vi "Repeat.vi"(11 "CSM Name":string="Repeat") -> ()   [LabVIEW 2026, in "UI-温度控制.lvlib" / "Repeat.lvlib"]
uses:
  Repeat.lvlib
  Supports/Repeat Steps.ctl
  Supports/Repeating States.ctl
  <userlib>/_NEVSTOP/Communicable State Machine(CSM)/_Polymophic/CSM - Filter Duplicated Lines.vi
  816fba94-53db-458f-9fde-c2796c7a1569.vi
  ba2d9a0e-10df-4741-bda9-2194bb22ae09.vi
  ed04b07b-11fd-4180-b0fa-2f6e8442eecc.vi
  <userlib>/_NEVSTOP/Communicable State Machine(CSM)/_Polymophic/Build Synchronous Message with Arguments.vi
  63e03b33-849f-44e3-ac5e-f4abb9122a72.vi
  801019de-d43e-4a0a-86cc-ff4224036546.vi
  2ffd62ee-fbfc-4690-b0a4-2e8231dd450f.vi
  1f220b95-32e7-4906-b34d-524106bf87b5.vi
  b2c443a6-884a-417f-a1f3-5b041c9b1280.vi
  <userlib>/_NEVSTOP/Communicable State Machine(CSM)/AdvanceAPI/CSM - Compact Multiple States.vi
  <userlib>/_NEVSTOP/Communicable State Machine(CSM)/AdvanceAPI/CSM - Break Down Multiple States String.vi
  <userlib>/_NEVSTOP/Communicable State Machine(CSM)/_Shared/Remove Comments from Single-line.vi
  <userlib>/_NEVSTOP/Communicable State Machine(CSM)/_Shared/Split Single-line Message.vi
  <userlib>/_NEVSTOP/Communicable State Machine(CSM)/_Shared/Trim Single-line Text.vi
  <userlib>/_NEVSTOP/Communicable State Machine(CSM)/AdvanceAPI/CSM - Revert Arguments-Safe String.vi
  <userlib>/_NEVSTOP/Communicable State Machine(CSM)/AdvanceAPI/CSM - Make String Arguments Safe.vi
  <userlib>/_NEVSTOP/Communicable State Machine(CSM)/_Support/Message/Parse State with Arguments String.vi
  <userlib>/_NEVSTOP/Communicable State Machine(CSM)/AdvanceAPI/CSM - Keywords.vi
  <userlib>/_NEVSTOP/Communicable State Machine(CSM)/addons/API-String-Arugments-Support/_Support/Convert API String Arguments to Data(variant).vi
  <userlib>/_NEVSTOP/Communicable State Machine(CSM)/addons/API-String-Arugments-Support/_Support/Data To API String Arguments.vi
  <userlib>/_NEVSTOP/Communicable State Machine(CSM)/Communicable State Machine.lvlib
  <userlib>/_NEVSTOP/Communicable State Machine(CSM)/addons/Loop-Support/CSM Loop Support.lvlib
  <userlib>/_NEVSTOP/Communicable State Machine(CSM)/addons/INI-Static-Variable-Support/INI-Static-Variable-Support.lvlib
panel:
  in  "运行次数":dbl=inf format="%#.0f"
  out "当前次数":i32
  in  "通道选择":enum32{"1", "2", "1&2"}(radio)
  in  "循环开始":bool
  in  "步骤":T1=[{"控制温度"=25.0, "时长(s)"=600.0, "进度"=0.0, "温控开关"=FALSE}, {"控制温度"=25.0, "时长(s)"=600.0, "进度"=0.0, "温控开关"=FALSE}, {"控制温度"=25.0, "时长(s)"=600.0, "进度"=0.0, "温控开关"=FALSE}, {"控制温度"=25.0, "时长(s)"=600.0, "进度"=0.0, "温控开关"=FALSE}] {"进度" scale=0.0..1.0; "控制温度" format="%.2g"}
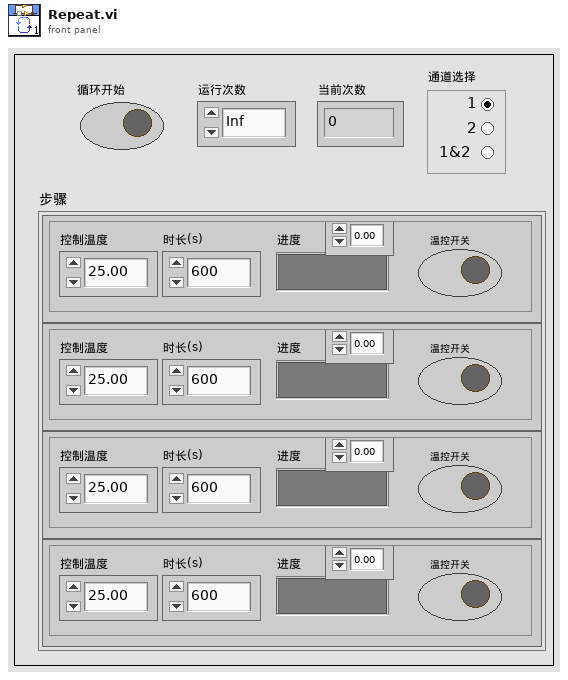
[diagram p1: front panel]
types:
  T1 = typedef "UI-温度控制.lvlib/Repeat Steps.ctl" = cluster{"控制温度":dbl, "时长(s)":dbl, "进度":dbl, "温控开关":bool}[]
  T2 = enum32{"Invalid", "Standard", "Closed", "Hidden", "Minimized", "Maximized"}
  T3 = enum32{"invalid app kind", "Development System", "Run Time System", "Student Edition", "Embedded LabVIEW", "Evaluation", "Custom"}
  T4 = typedef "UI-温度控制.lvlib/Repeat.lvlib/Repeating States.ctl" = enum16{"Idle", "Repeating", "Error"}
  T5 = typedef "Communicable State Machine.lvlib/_CSM_Response Source Message.ctl" = cluster{"‘State":string, "’Arguments":string, "’Error":errorcluster}
  T6 = cluster{"Current VI Reference":refnum<vi>, "Close Panel on Exit?":bool}
  T7 = cluster{"Core":cluster{"Current VI Reference":refnum<vi>, "Close Panel on Exit?":bool}, "State":T4, "Repeat":cluster{"温控步骤开始时间":timestamp, "温控步骤索引":i32[], "下一步？":bool}, "CSM Name":string, "INI Path":path}
  T8 = cluster{"温控步骤开始时间":timestamp, "温控步骤索引":i32[], "下一步？":bool}
  T9 = cluster{"控制温度":dbl, "时长(s)":dbl, "进度":dbl, "温控开关":bool}
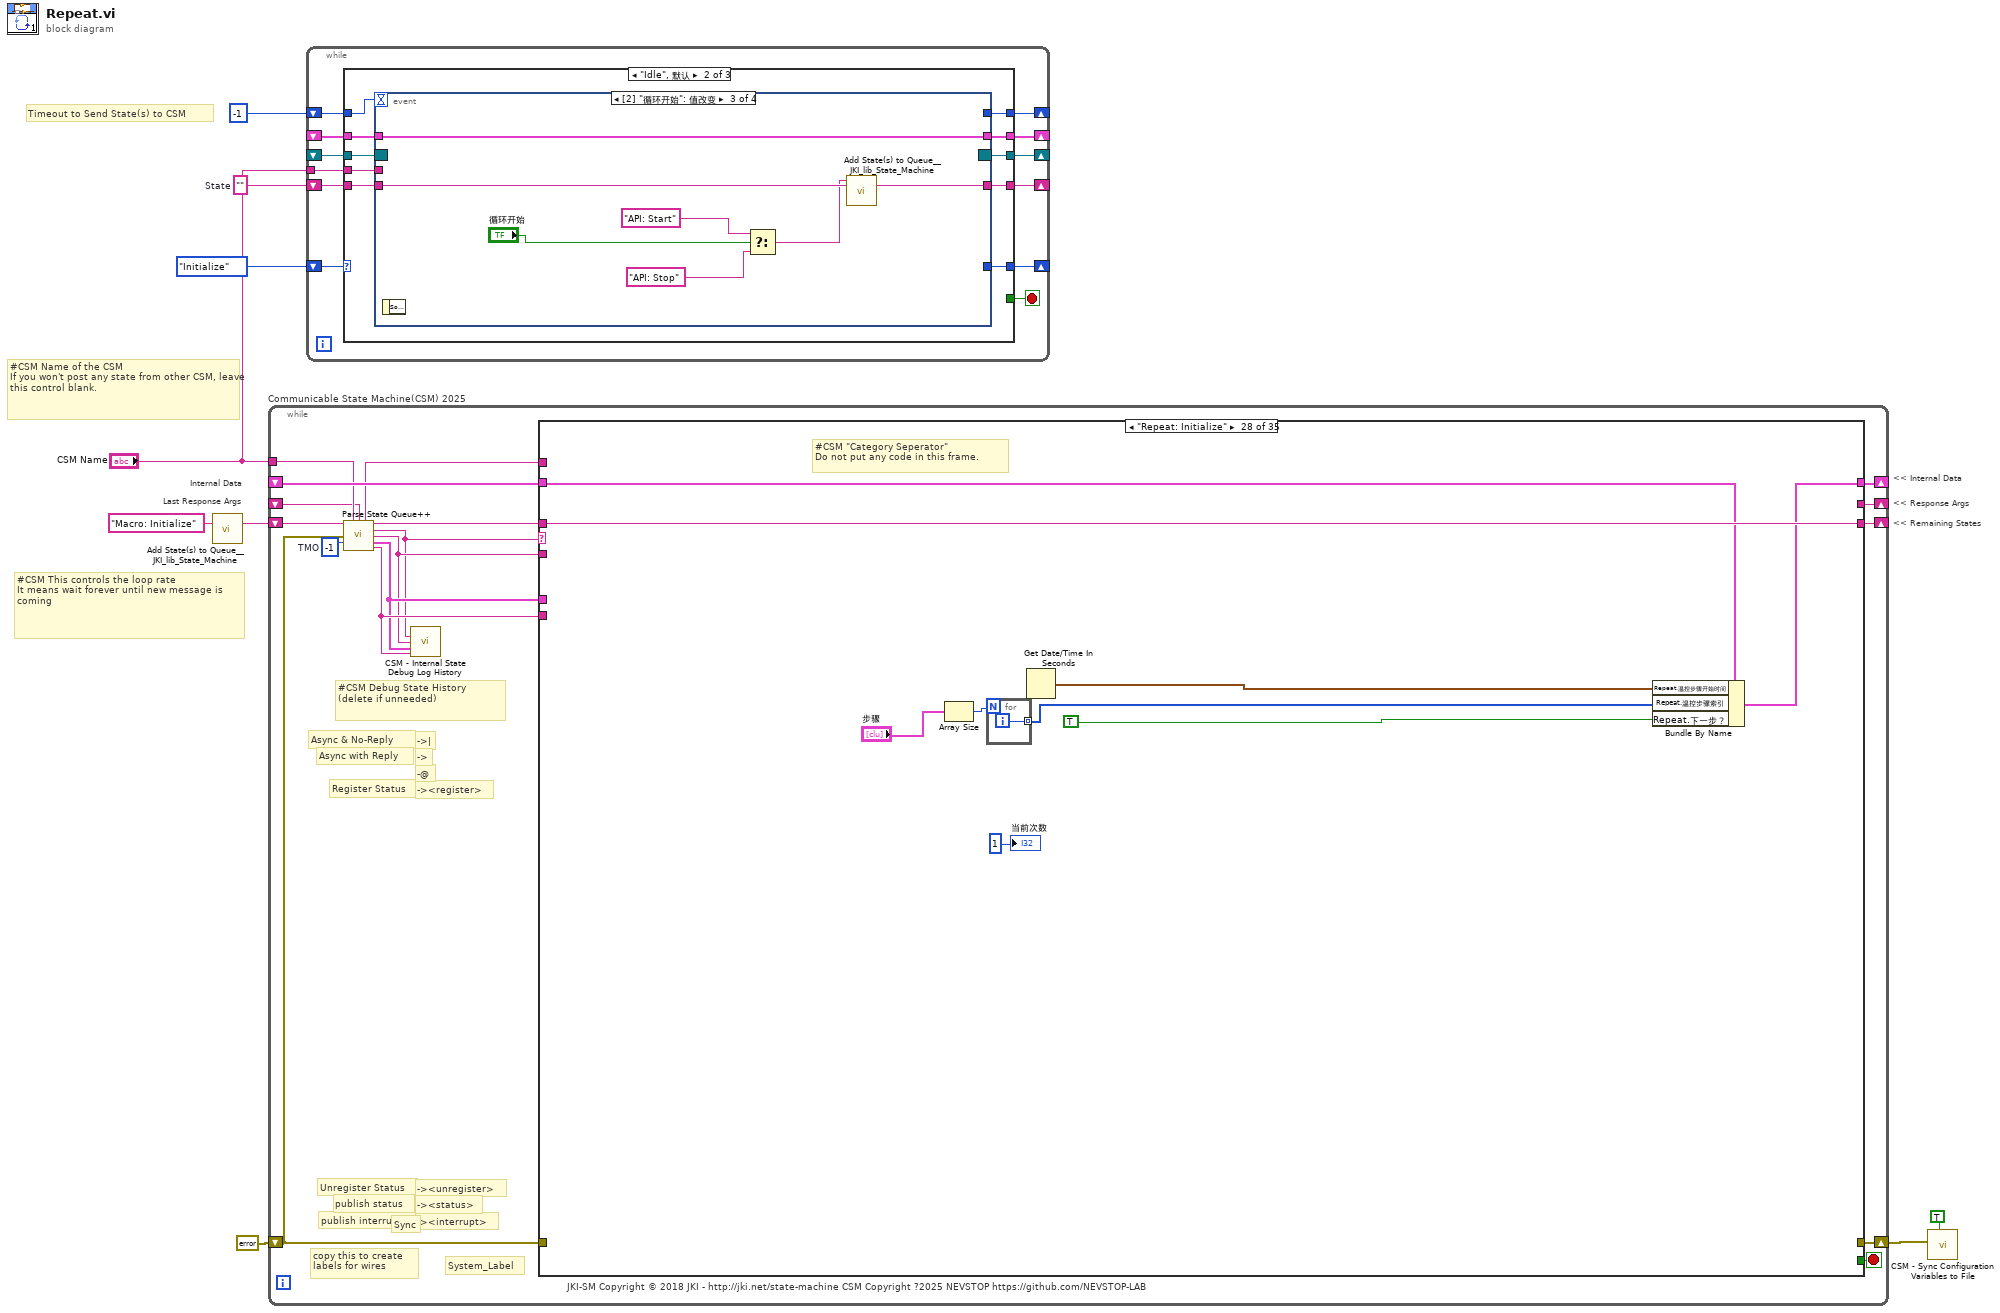
[diagram p0: block diagram]
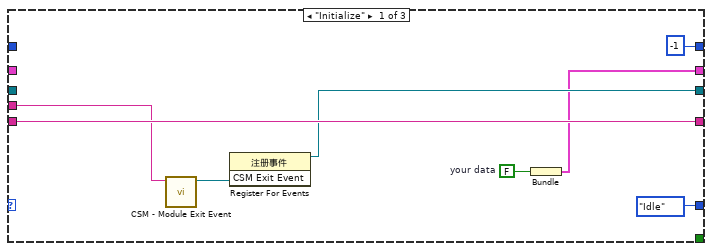
[diagram p2: hidden frame]
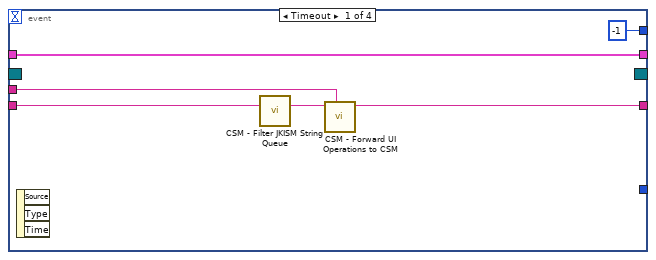
[diagram p3: hidden frame]
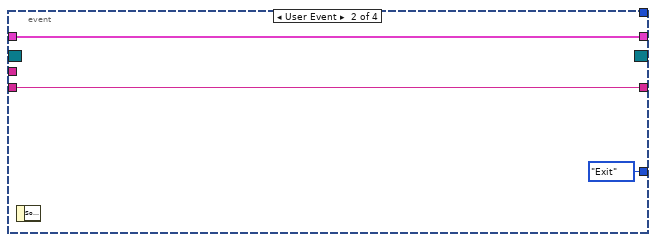
[diagram p4: hidden frame]
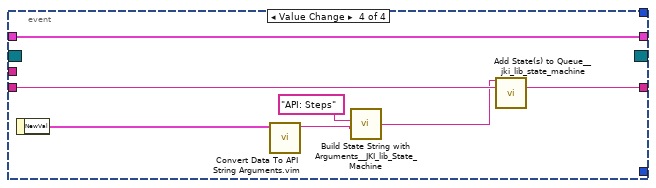
[diagram p5: hidden frame]
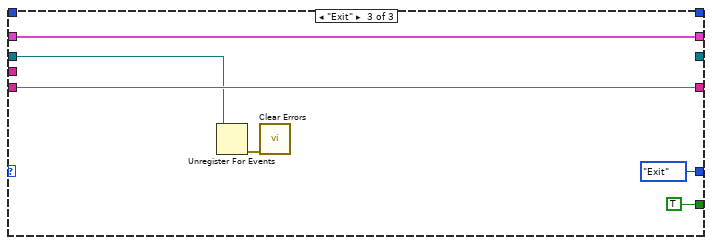
[diagram p6: hidden frame]
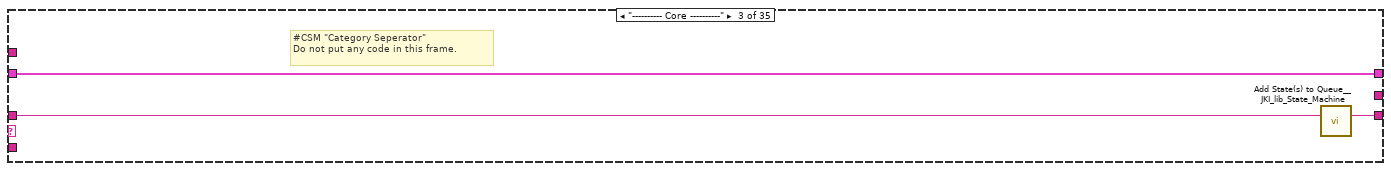
[diagram p9: hidden frame]
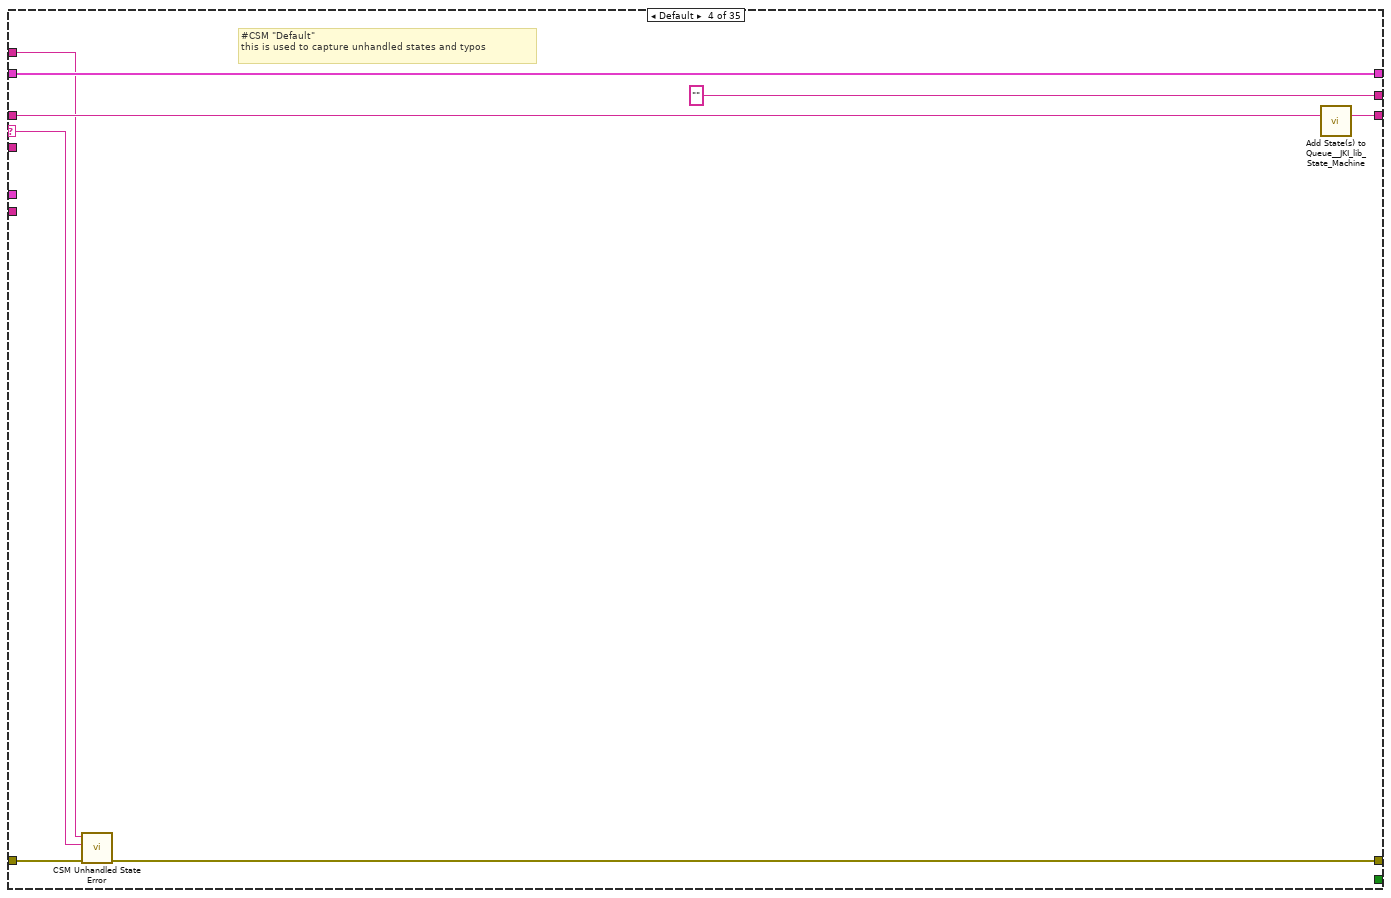
[diagram p10: hidden frame]
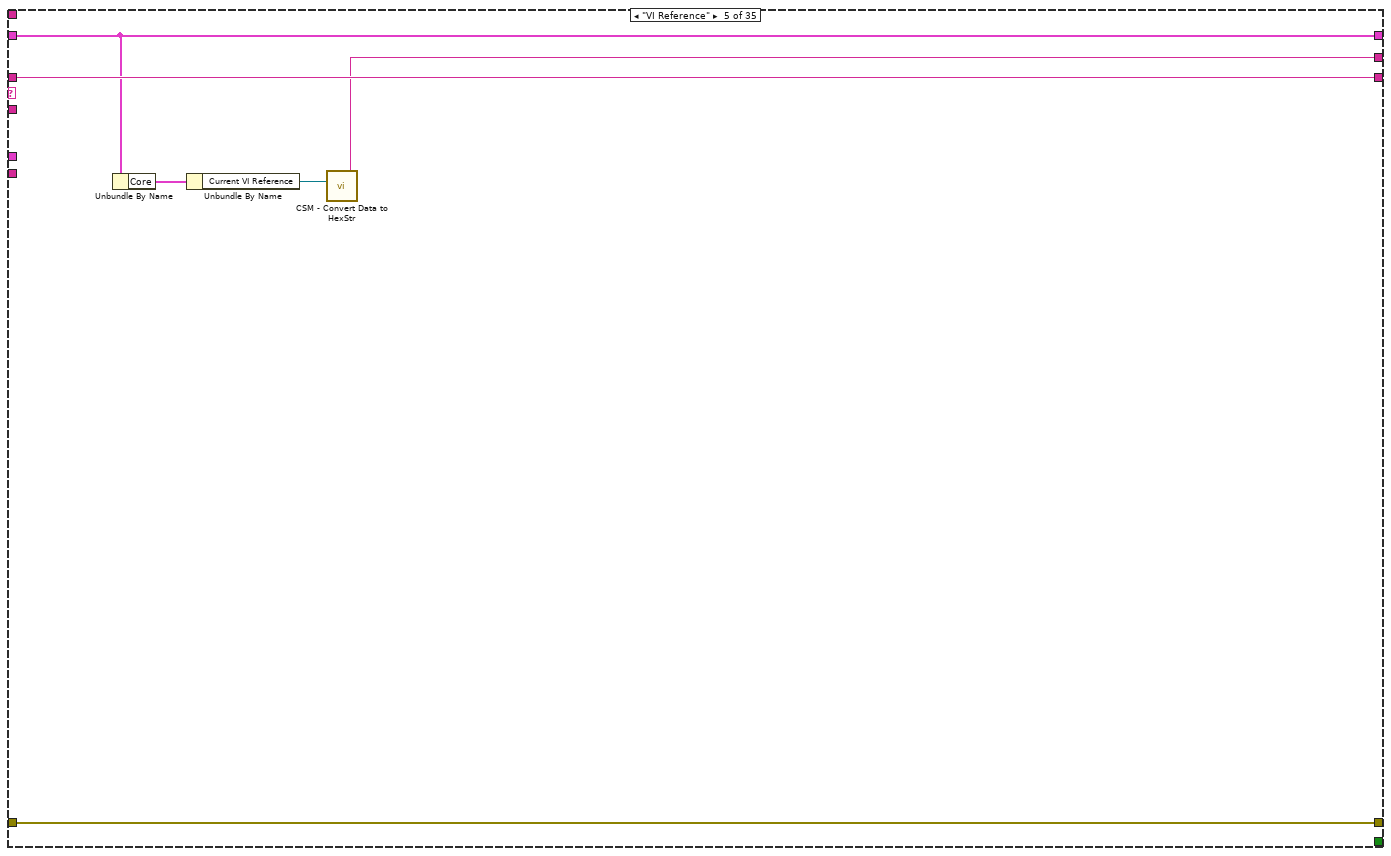
[diagram p11: hidden frame]
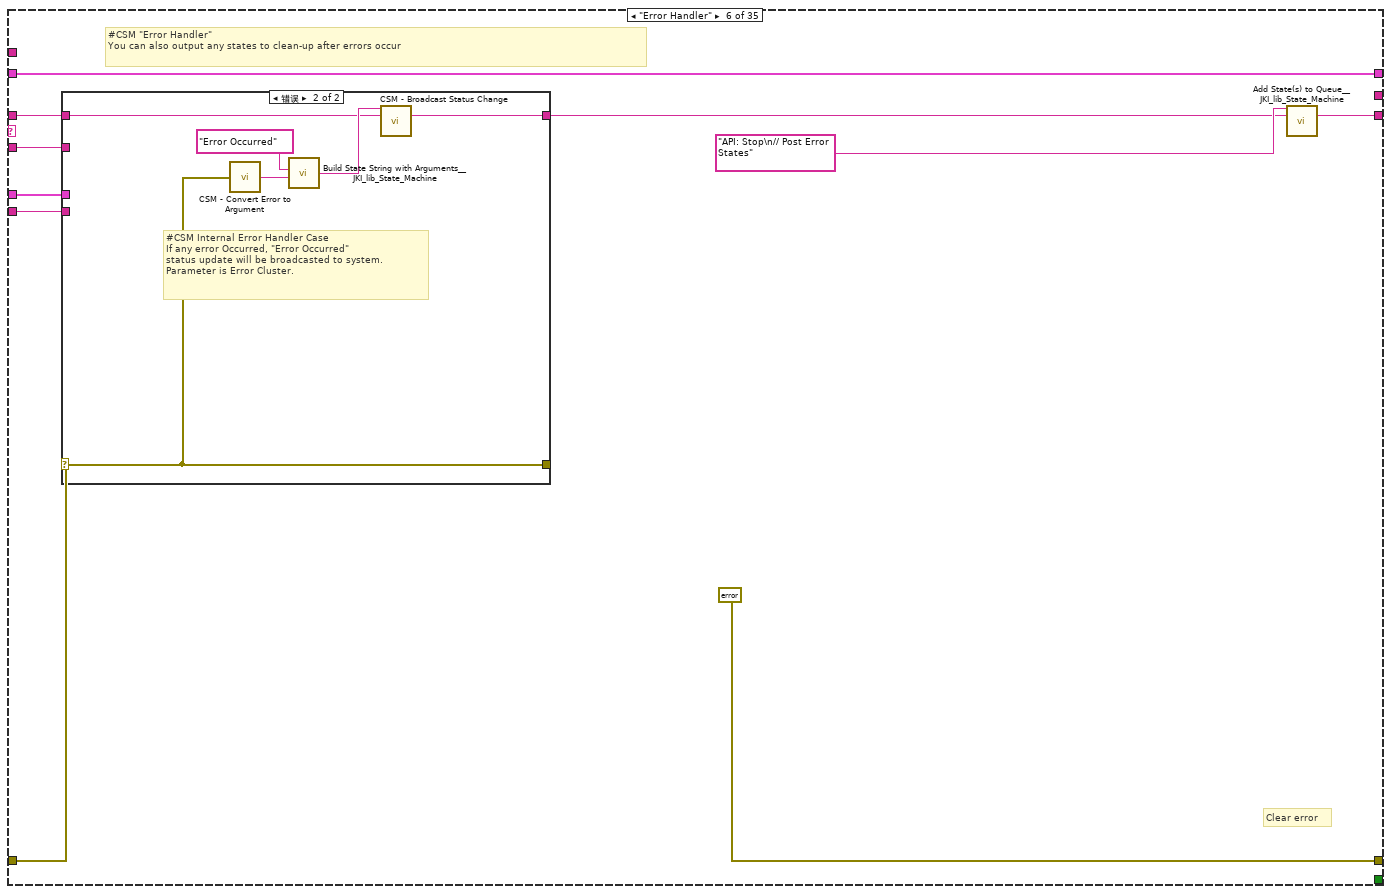
[diagram p12: hidden frame]
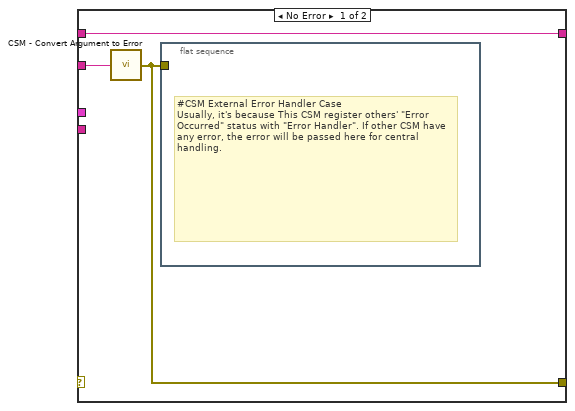
[diagram p13: hidden frame]
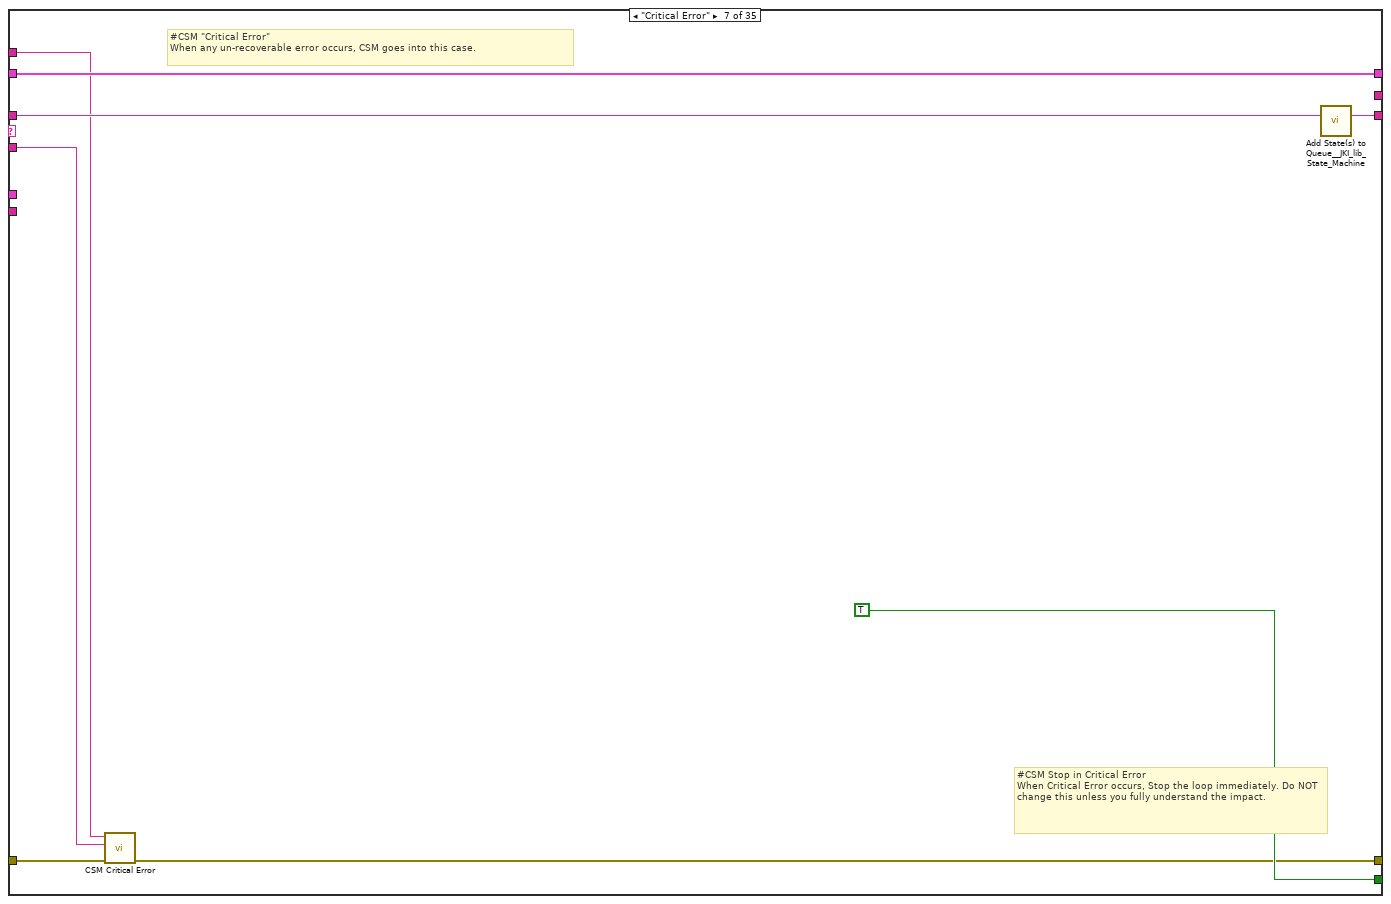
[diagram p14: hidden frame]
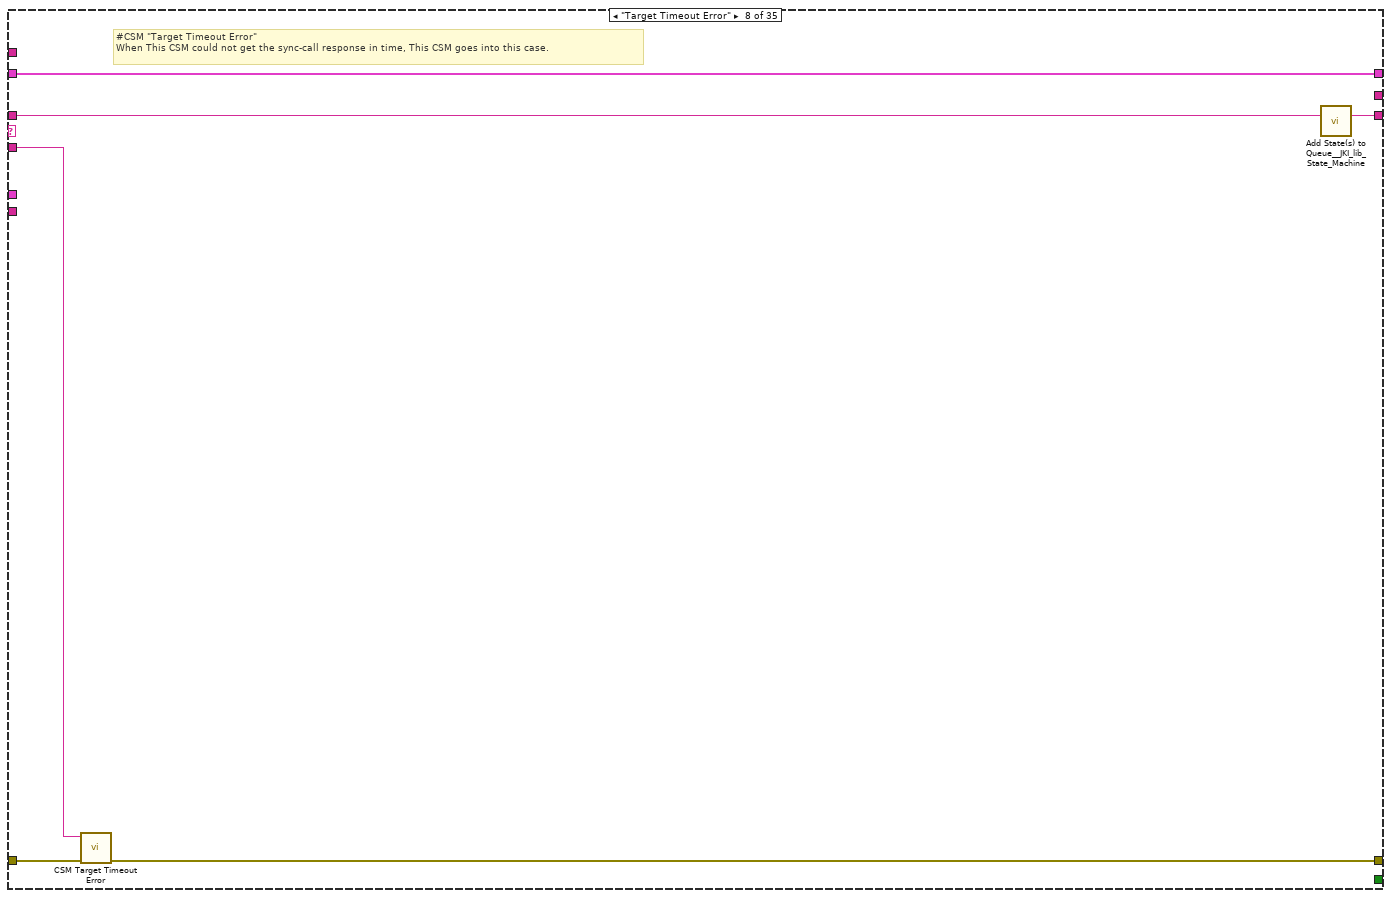
[diagram p15: hidden frame]
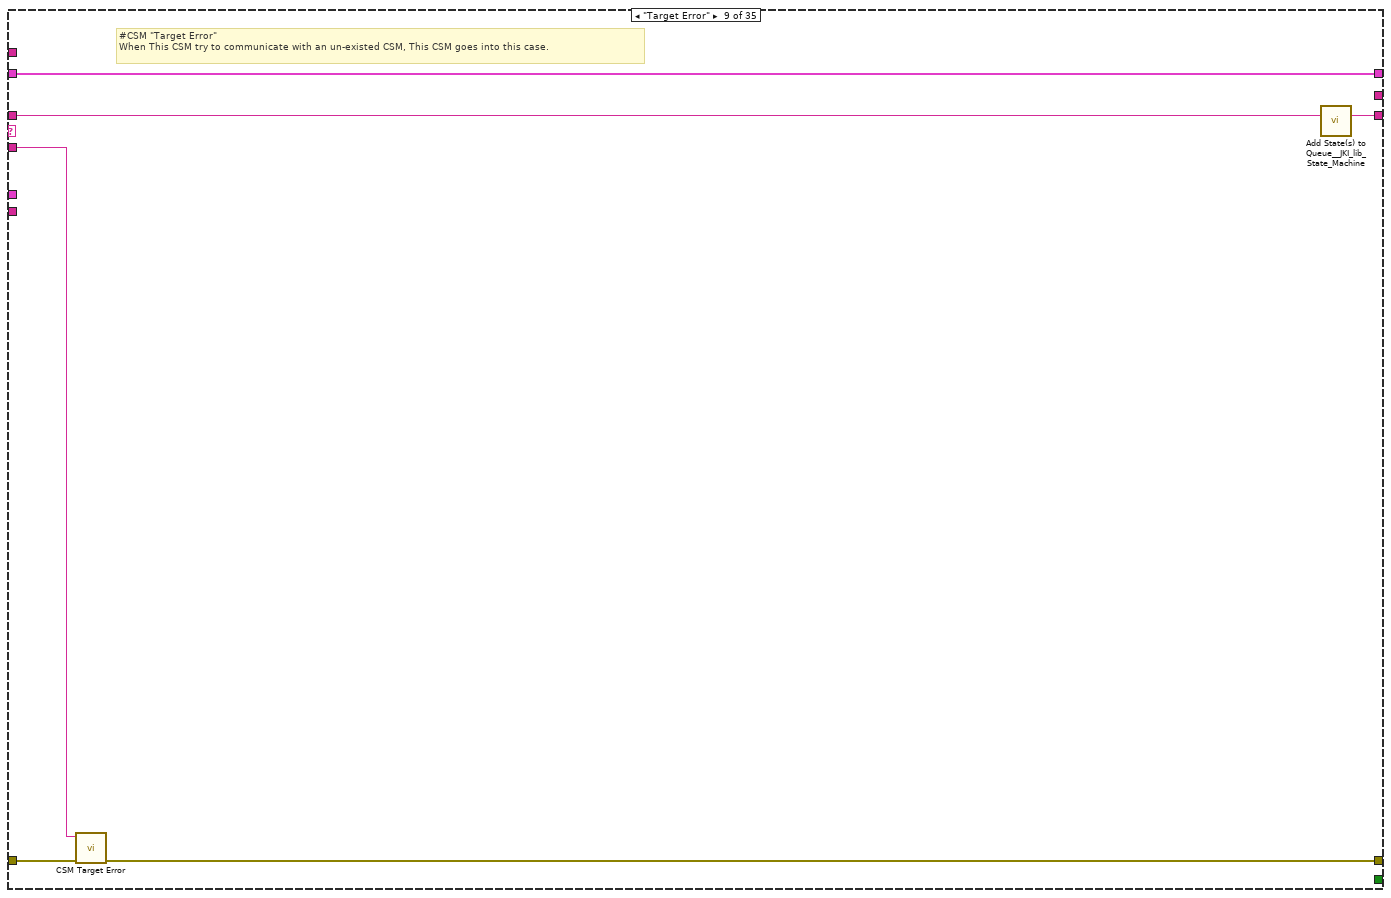
[diagram p16: hidden frame]
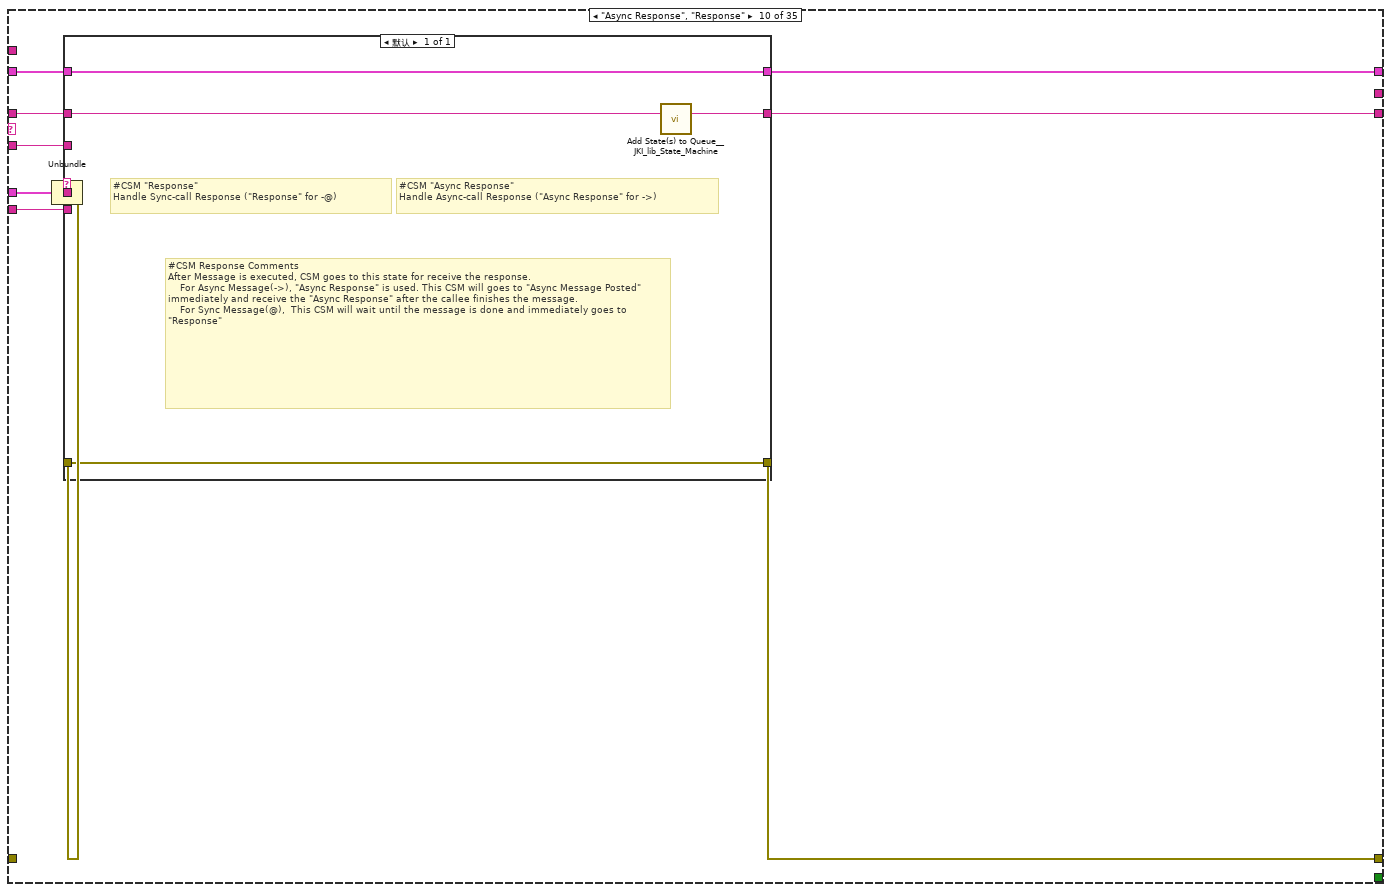
[diagram p17: hidden frame]
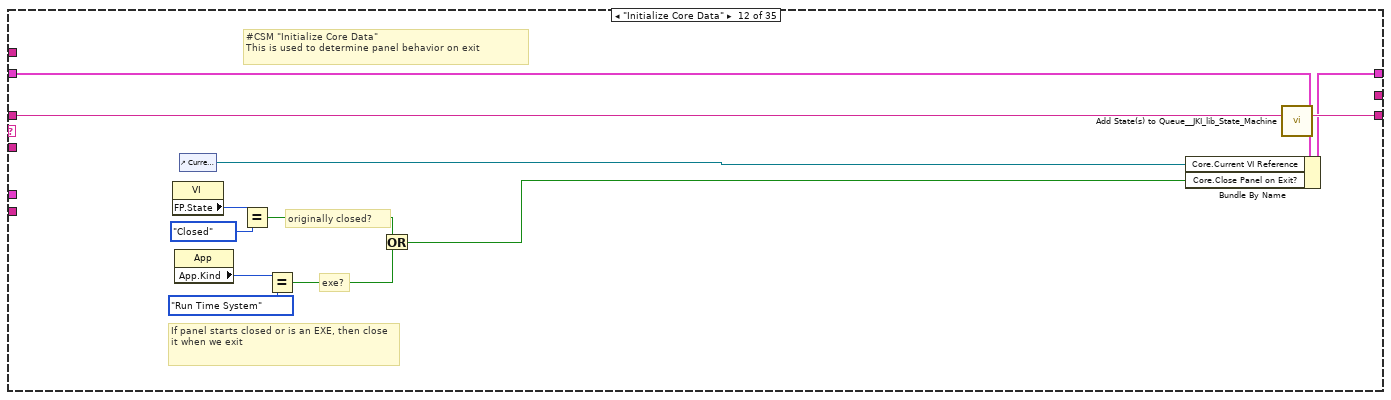
[diagram p19: hidden frame]
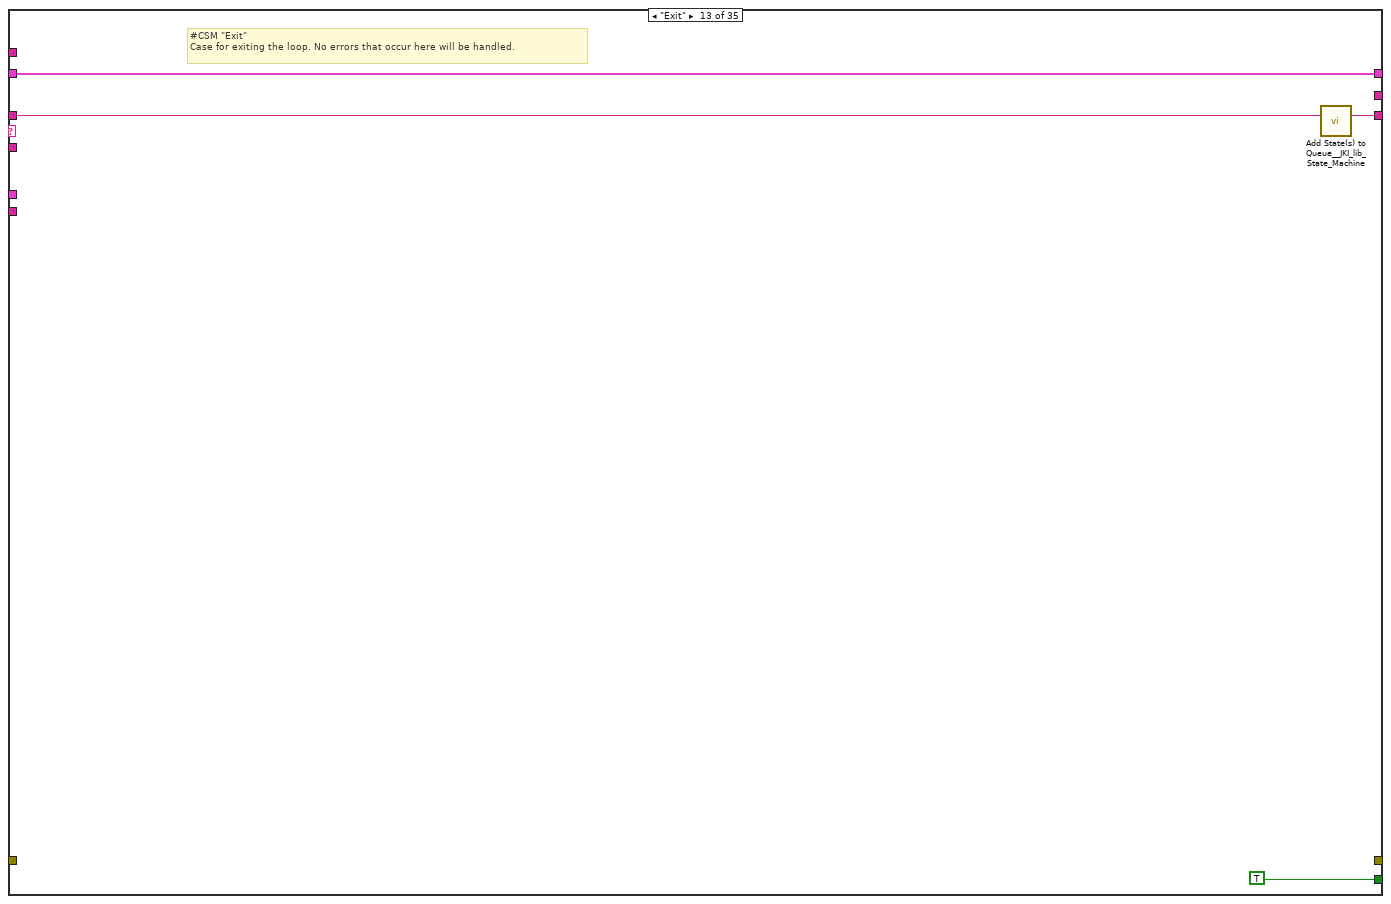
[diagram p20: hidden frame]
diagram:
  w5 = ""  # State
  # "Timeout to Send State(s) to CSM"
  # "Last Response Args"
  # "Internal Data"
  # "#CSM Name of the CSM\nIf you won't post any state from other CSM, leave this control blank."
  # "#CSM This controls the loop rate\nIt means wait forever until new message is coming"
  # "<< Internal Data"
  # "<< Response Args"
  # "<< Remaining States"
  n1 = call <vilib>:"Add State(s) to Queue__JKI_lib_State_Machine.vi"("State(s) in (\"\")"="Macro: Initialize" ("Init State(\"Macro: Initialize\")")) -> ("States Out"=w7:string)  [unwired: 14 in]
  n2 = while "Communicable State Machine(CSM) 2025" {
    shift-right: [w21] -> _
    shift-left: _ -> [w20]
    shift-right: [w24] -> w2
    shift-left: errorcluster {"status"=FALSE, "code"=0, "source"=""} ("error out") -> [w10]
    shift-right: [w23] -> _
    shift-left: w7 -> [w25]
    tunnel: "CSM Name" -> [w17]
    shift-right: [w18] -> _
    shift-left: _ -> [w12]
    stop <- w22 stop-if-true
    w19 = -1  # TMO
    # "#CSM Debug State History\n(delete if unneeded)"
    # "-><interrupt>"
    # "-><status>"
    # "-><unregister>"
    # "-><register>"
    # "-@"
    # "->"
    # "->|"
    # "publish interrupt"
    # "publish status"
    # "Unregister Status"
    # "Register Status"
    # "Sync"
    # "Async with Reply"
    # "Async & No-Reply"
    # "JKI-SM Copyright © 2018 JKI - http://jki.net/state-machine CSM Copyright ?2025 NEVSTOP https://github.com/NEVSTOP-LAB"
    # "copy this to create labels for wires"
    # "System_Label"
    n3 = call <userlib>:"Parse State Queue++.vi"("State Queue"=w25, "Name (\"\" to Use UUID)"=w17, "Response Arguments"=w12, "Previous Error"=w10, "Dequeue (1 ms)"=w19) -> ("Name Used"=w11:string, "Remaining States"=w26:string, "Current State"=w13:string, "Arguments"=w14:string, "Additional Information"=w15:T5, "Source CSM"=w16:string)  [unwired: 5 in]
    n4 = call <userlib>:"CSM - Internal State Debug Log History.vi"("State"=w13, "Arguments (\"\")"=w14, ">> Response Source Message >>"=w15, "Source (\"\")"=w16) -> ()  [unwired: 11 in, 1 out]
    n5 = case shown="\"Repeat: Initialize\"" w13 {
      selector: w13 -> [_ _ _ w37 _ _ _ _ _ _ _ _ _ _ _ _ _ _ _ _ _ _ _ _ _ _ _ _ _ _ _ _ _ w342 _]
      tunnel: w26 -> [w27 w30 w33 w41 w46 w51 w74 w80 w86 w96 w103 w115 w119 w122 w130 w133 w139 w142 w146 w154 w159 w163 w174 w181 w185 w194 w198 w207 w210 w264 w330 w335 w338 w343 w347]
      tunnel: w14 -> [_ _ _ _ _ w50 w70 w77 w83 w90 _ _ _ _ _ _ _ _ _ _ _ _ _ w180 w183 w192 _ _ _ _ _ _ _ w340 _]
      tunnel: w20 -> [w28 w29 w31 w39 w45 w56 w72 w78 w84 w94 w102 w109 w117 w120 _ w132 w135 w140 w144 w147 w160 w161 w175 w179 w188 w193 w196 w205 w215 w269 w328 w333 w336 w344 w346]
      tunnel: [_ _ _ w34 w47 errorcluster {"status"=FALSE, "code"=0, "source"=""} ("error out") w67 w75 w81 w97 _ _ _ _ _ _ w136 _ _ _ _ _ _ w182 w189 w195 _ _ w212 w283 _ _ _ _ w348] -> w24
      tunnel: w10 -> [_ _ _ w35 w47 w54 w68 w76 w82 _ _ _ _ _ _ _ w134 _ _ _ _ _ _ w182 w189 w195 _ _ w214 w283 _ _ _ _ w348]
      tunnel: [w27 w30 w32 w40 w46 w52 w73 w79 w85 w95 w103 w114 w118 w121 w129 w133 w138 w141 w145 w153 w158 w162 w173 w181 w184 w194 w197 w207 w211 w265 w329 w334 w337 w341 w345] -> w23
      tunnel: [_ _ _ _ _ _ TRUE _ _ _ _ _ TRUE _ _ _ _ _ _ _ _ _ _ _ _ _ _ _ _ _ _ _ _ _ _] -> w22
      tunnel: [w28 w29 w31 w39 w45 w56 w72 w78 w84 w93 w102 w113 w117 w120 w128 w132 w135 w140 w144 w147 w160 w164 w175 w178 w188 w193 w196 w206 w213 w268 w328 w332 w336 w344 w346] -> w21
      tunnel: w16 -> [_ _ _ _ _ w49 _ _ _ w91 _ _ _ _ _ _ _ _ _ _ _ _ _ _ _ _ _ _ _ _ _ _ _ _ _]
      tunnel: w15 -> [_ _ _ _ _ w48 _ _ _ w92 _ _ _ _ _ _ _ _ _ _ _ _ _ _ _ _ _ _ _ _ _ _ _ _ _]
      tunnel: [_ _ _ "" w42 _ _ _ _ _ _ _ _ _ _ _ _ _ _ _ _ _ _ _ _ _ _ _ _ _ _ _ _ _ _] -> w18
      tunnel: w11 -> [_ _ _ w36 _ _ w69 _ _ _ _ _ _ _ _ _ _ _ _ _ _ _ _ _ _ _ _ _ _ _ _ _ _ _ _]
      frame "", "Idle" {
        # "#CSM \"Idle/Event Handler\"\nexecutes when the state queue is empty"
      }
      frame "CSM Documentation" {
        # "#CSM State Syntax\n\n// Comment line, all text to the right of “//” will be ignored\n// Local Message Example\nDoSth: DoA >> Arguments\n\n// Sync Call Example\nAPI: xxxx >> Arguments -@ TargetModule\n\n// Async Call Example\nAPI: xxxx >> Arguments -> TargetModule\n\n// Async Call without Reply Example\nAPI: xxxx >> Arguments ->| TargetModule\n\n// Broadcast normal status:\nStatus >> StatusArguments  -><status>\n\n// Broadcast Interrupt status:\nInterrupt >> StatusArguments  -><interrupt>\n\n// Register Source Module's status to Handler Module\nStatus@Source Module >> Handler Module@Handler Module -><register>\n\n// Unegister Source Module's status\nStatus@Source Module >> Handler Module -><unregister>"
        # "#CSM README FIRST\n\nCommunicable State Machine(CSM) is a LabVIEW application framework that builds upon JKI State Machine(JKISM). It follows the pattern of JKISM and extends the keywords to describe message communication between modules, including concepts such as Sync-Message, Async-Message, Subscription/Unsubscription of status - essential elements for creating reusable code modules. For more information, please visit the CSM wiki: https://nevstop-lab.github.io/CSM-Wiki/\n\nFor instructions on JKI State Machine, visit: \n    http://jki.net/state-machine/\nFor information about CSM, visit: \n    https://github.com/NEVSTOP-LAB"
        # "#CSM \"Documentation\"\nCase for holding CSM Documenation"
      }
      frame "---------- Core ----------" {
        # "#CSM \"Category Seperator\"\nDo not put any code in this frame."
        n6 = call <vilib>:"Add State(s) to Queue__JKI_lib_State_Machine.vi"("State(s) in (\"\")"=w33) -> ("States Out"=w32:string)  [unwired: 14 in]
      }
      frame Default {
        # "#CSM \"Default\"\nthis is used to capture unhandled states and typos"
        n7 = call <userlib>:"CSM Unhandled State Error.vi"("error in (no error)"=w35, "Undefined State"=w37, "CSM Name"=w36) -> ("error out"=w34:errorcluster)  [unwired: 8 in]
        n8 = call <vilib>:"Add State(s) to Queue__JKI_lib_State_Machine.vi"("State(s) in (\"\")"=w41) -> ("States Out"=w40:string)  [unwired: 14 in]
      }
      frame "VI Reference" {
        n9 = Unbundle By Name(w45) -> ("Core"=w44:T6)
        n10 = Unbundle By Name(w44) -> ("Current VI Reference"=w43:refnum<vi>)
        n11 = call <userlib>:"CSM - Convert Data to HexStr.vi"("Variant"=w43) -> ("HEX String (0-9,A-F)"=w42:string)  [unwired: 8 in]
      }
      frame "Error Handler" {
        # "#CSM \"Error Handler\"\nYou can also output any states to clean-up after errors occur"
        # "Clear error"
        n12 = case shown="错误" w54 {
          selector: w54 -> [_ w61]
          tunnel: [w60 w63] -> w53
          tunnel: w51 -> [w60 w62]
          tunnel: w50 -> [w59 _]
          tunnel: w49 -> [_ _]
          tunnel: w48 -> [_ _]
          tunnel: [w58 w61] -> _
          frame No Error {
            n13 = call <userlib>:"CSM - Convert Argument to Error.vi"("Argument"=w59) -> ("Error"=w58:errorcluster)  [unwired: 4 in]
            n14 = flat-sequence {
              tunnel: w58 -> [_]
              frame #0 {
                # "#CSM External Error Handler Case\nUsually, it's because This CSM register others' \"Error Occurred\" status with \"Error Handler\". If other CSM have any error, the error will be passed here for central handling."
              }
            }
          }
          frame Error {
            # "#CSM Internal Error Handler Case \nIf any error Occurred, \"Error Occurred\" \nstatus update will be broadcasted to system.\nParameter is Error Cluster."
            n15 = call <userlib>:"CSM - Convert Error to Argument.vi"("Error"=w61) -> ("Argument"=w65:string)  [unwired: 4 in]
            n16 = call <vilib>:"Build State String with Arguments__JKI_lib_State_Machine.vi"("Arguments (\"\")"=w65, "State"="Error Occurred" ("Status with Arguments")) -> ("State with Arguments"=w64:string)  [unwired: 4 in]
            n17 = call <userlib>:"CSM - Broadcast Status Change.vi"("Status With Arguments"=w64, "State Queue"=w62) -> ("Remaining States"=w63:string)  [unwired: 13 in]
          }
        }
        n18 = call <vilib>:"Add State(s) to Queue__JKI_lib_State_Machine.vi"("State(s) in Front (\"\")"="API: Stop\n// Post Error States", "State(s) in (\"\")"=w53) -> ("States Out"=w52:string)  [unwired: 13 in]
      }
      frame "Critical Error" {
        # "#CSM \"Critical Error\"\nWhen any un-recoverable error occurs, CSM goes into this case."
        # "#CSM Stop in Critical Error\nWhen Critical Error occurs, Stop the loop immediately. Do NOT change this unless you fully understand the impact."
        n19 = call <userlib>:"CSM Critical Error.vi"("error in (no error)"=w68, "Arugments (As Reason)"=w70, "CSM Name"=w69) -> ("error out"=w67:errorcluster)  [unwired: 8 in]
        n20 = call <vilib>:"Add State(s) to Queue__JKI_lib_State_Machine.vi"("State(s) in (\"\")"=w74) -> ("States Out"=w73:string)  [unwired: 14 in]
      }
      frame "Target Timeout Error" {
        # "#CSM \"Target Timeout Error\"\nWhen This CSM could not get the sync-call response in time, This CSM goes into this case."
        n21 = call <userlib>:"CSM Target Timeout Error.vi"("error in (no error)"=w76, "Arguments (As CSM Name)"=w77) -> ("error out"=w75:errorcluster)  [unwired: 9 in]
        n22 = call <vilib>:"Add State(s) to Queue__JKI_lib_State_Machine.vi"("State(s) in (\"\")"=w80) -> ("States Out"=w79:string)  [unwired: 14 in]
      }
      frame "Target Error" {
        # "#CSM \"Target Error\"\nWhen This CSM try to communicate with an un-existed CSM, This CSM goes into this case."
        n23 = call <userlib>:"CSM Target Error.vi"("error in (no error)"=w82, "Arguments (As CSM Name)"=w83) -> ("error out"=w81:errorcluster)  [unwired: 9 in]
        n24 = call <vilib>:"Add State(s) to Queue__JKI_lib_State_Machine.vi"("State(s) in (\"\")"=w86) -> ("States Out"=w85:string)  [unwired: 14 in]
      }
      frame "Async Response", "Response" {
        n25 = Unbundle(w92) -> ("‘State"=w89:string, "’Arguments"=w88:string, "’Error"=w87:errorcluster)
        n26 = case shown="默认" w89 {
          tunnel: [w98] -> w95
          tunnel: w96 -> [w99]
          tunnel: [w101] -> w93
          tunnel: w94 -> [w101]
          tunnel: [w100] -> w97
          tunnel: w87 -> [w100]
          tunnel: w91 -> [_]
          tunnel: w90 -> [_]
          tunnel: w88 -> [_]
          frame 默认 {
            # "#CSM \"Async Response\"\nHandle Async-call Response (\"Async Response\" for ->)"
            # "#CSM \"Response\"\nHandle Sync-call Response (\"Response\" for -@)"
            # "#CSM Response Comments\nAfter Message is executed, CSM goes to this state for receive the response.\n    For Async Message(->), \"Async Response\" is used. This CSM will goes to \"Async Message Posted\" immediately and receive the \"Async Response\" after the callee finishes the message.\n    For Sync Message(@),  This CSM will wait until the message is done and immediately goes to \"Response\""
            n27 = call <vilib>:"Add State(s) to Queue__JKI_lib_State_Machine.vi"("State(s) in (\"\")"=w99) -> ("States Out"=w98:string)  [unwired: 14 in]
          }
        }
      }
      frame "Async Message Posted" {
        # "#CSM \"Async Message Posted\"\nAfter Async Message is posted (-> or ->| ), CSM goes to this state for post-action.\nYou can use Argument - State to tell which Async Message is called."
      }
      frame "Initialize Core Data" {
        # "#CSM \"Initialize Core Data\"\nThis is used to determine panel behavior on exit"
        # "originally closed?"
        # "exe?"
        # "If panel starts closed or is an EXE, then close it when we exit"
        n28 = property class="VI"() -> ("FP.State"=w106:T2)  [unwired: 2 in, 2 out]
        n29 = property class="App"() -> ("App.Kind"=w112:T3)  [unwired: 2 in, 2 out]
        n30 = control-ref of="Current VI Reference"() -> (w107:refnum<vi>)
        n31 = Equal?(x=w106, y=T2."Closed" ("Front Panel Window:State")) -> (x = y?=w104:bool)
        n32 = Equal?(x=w112, y=T3."Run Time System" ("Application:Kind")) -> (x = y?=w110:bool)
        n33 = Or(x=w104, y=w110) -> (x .or. y?=w108:bool)
        n34 = Bundle By Name(cluster=w109, "Core.Current VI Reference"=w107, "Core.Close Panel on Exit?"=w108) -> (w113:T7)
        n35 = call <vilib>:"Add State(s) to Queue__JKI_lib_State_Machine.vi"("State(s) in (\"\")"=w115) -> ("States Out"=w114:string)  [unwired: 14 in]
      }
      frame "Exit" {
        # "#CSM \"Exit\"\nCase for exiting the loop. No errors that occur here will be handled."
        n36 = call <vilib>:"Add State(s) to Queue__JKI_lib_State_Machine.vi"("State(s) in (\"\")"=w119) -> ("States Out"=w118:string)  [unwired: 14 in]
      }
      frame "---------- Data ----------" {
        # "#CSM \"Category Seperator\"\nDo not put any code in this frame."
        n37 = call <vilib>:"Add State(s) to Queue__JKI_lib_State_Machine.vi"("State(s) in (\"\")"=w122) -> ("States Out"=w121:string)  [unwired: 14 in]
      }
      frame "Data: Initialize" {
        w123 = path ""  # INI Path
        w125 = ""  # CSM Name
        w124 = T8 {"温控步骤开始时间"=timestamp(0 s since 1904-01-01), "温控步骤索引"=[0, 1, 2, 3], "下一步？"=FALSE}  # Repeat
        w126 = Repeating_States."Idle"  # State
        w127 = T6 {"Current VI Reference"=refnum, "Close Panel on Exit?"=FALSE}  # Core
        # "#CSM \"Data: Initialize\"\nInitialize the shift-register data, here.\n(data names are defined by what you wire into the bundle function)"
        # "#CSM do not delete - used by framework"
        # "#CSM Data names and types of shift register data are defined by this bundle."
        n38 = Bundle("Core"=w127, "State"=w126, "Repeat"=w124, "CSM Name"=w125, "INI Path"=w123) -> (w128:T7)  [unwired: 1 in]
        n39 = call <vilib>:"Add State(s) to Queue__JKI_lib_State_Machine.vi"("State(s) in (\"\")"=w130) -> ("States Out"=w129:string)  [unwired: 14 in]
      }
      frame "Data: Update Indicators" {
        n40 = local write "循环开始"(FALSE ("循环开始")) -> ()
      }
      frame "Data: Cleanup" {
        # "#CSM \"Data: Cleanup\"\nCleanup any data and references, here.\n(this is called automatically, by the Macro: Exit)"
        n41 = Unbundle By Name(w135) -> ("Core.Current VI Reference"=w137:refnum<vi>)
        n42 = Close Reference(reference=w137, error in (no error)=w134) -> (error out=w136:errorcluster)
        n43 = call <vilib>:"Add State(s) to Queue__JKI_lib_State_Machine.vi"("State(s) in (\"\")"=w139) -> ("States Out"=w138:string)  [unwired: 14 in]
      }
      frame "---------- Macro ----------" {
        # "#CSM \"Category Seperator\"\nDo not put any code in this frame."
        n44 = call <vilib>:"Add State(s) to Queue__JKI_lib_State_Machine.vi"("State(s) in (\"\")"=w142) -> ("States Out"=w141:string)  [unwired: 14 in]
      }
      frame "Macro: Initialize" {
        # "#CSM \"Macro: Initialize\"\nInitialization Macro (This is called once, when the VI starts)"
        n45 = call <vilib>:"Add State(s) to Queue__JKI_lib_State_Machine.vi"("State(s) in Front (\"\")"="Data: Initialize\nInitialize Core Data\nData: Update Indicators", "State(s) in (\"\")"=w146) -> ("States Out"=w145:string)  [unwired: 13 in]
      }
      frame "Macro: Exit" {
        # "#CSM \"Macro: Exit\"\nExit Macro (This is called once, when the VI exits)"
        n46 = Unbundle By Name(w147) -> ("State"=w151:T4)
        n47 = case shown="\"Repeating\"" w151 {
          tunnel: ["" "Break Continuous\nRepeat: Close" ""] -> w149
          frame "Idle", Default {
          }
          frame "Repeating" {
          }
          frame "Error" {
          }
        }
        n48 = call <vilib>:"Add State(s) to Queue__JKI_lib_State_Machine.vi"("State(s) in Front (\"\")"="//Exit Sub-Modules ", "State(s) in (\"\")"=w149, "State(s) at Back (\"\")"="Data: Cleanup\nExit") -> ("States Out"=w148:string)  [unwired: 12 in]
        n49 = call <vilib>:"Add State(s) to Queue__JKI_lib_State_Machine.vi"("State(s) in Front (\"\")"=w148, "State(s) in (\"\")"=w154) -> ("States Out"=w153:string)  [unwired: 13 in]
      }
      frame "---------- API ----------" {
        # "#CSM \"Category Seperator\"\nDo not put any code in this frame."
        n50 = call <vilib>:"Add State(s) to Queue__JKI_lib_State_Machine.vi"("State(s) in (\"\")"=w159) -> ("States Out"=w158:string)  [unwired: 14 in]
      }
      frame "API: Start" {
        # "#CSM API Example\nCopy/Rename this case for your own API"
        n51 = Unbundle By Name(w161) -> ("State"=w166:T4)
        n52 = case shown="\"Idle\"" w166 {
          selector: w166 -> [_ w170 w171]
          tunnel: [Repeating_States."Repeating" ("Acquisition State") w170 w171] -> w167
          tunnel: ["Repeat: Initialize \nRepeat: Judge\nContinuous Check >> Repeat: Judge -><loop> \nRepeat: Stop\nRepeat: Close " ("State(s) in Front (\"\")") _ _] -> w165
          frame "Idle" {
            # "If the system is idle, start the acquisition."
          }
          frame "Repeating" {
            # "The system is already acquiring. Ignore the \"Start\" message."
          }
          frame "Error" {
          }
        }
        n53 = call <userlib>:"CSMLS - Define Loop State(s).vi"("Loop States"=w165, "States Queue"=w163) -> ("Remaining States"=w162:string)  [unwired: 13 in]
        n54 = Bundle By Name(cluster=w161, "State"=w167) -> (w164:T7)
      }
      frame "API: Stop" {
        # "#CSM API Example\nCopy/Rename this case for your own API"
        n55 = Unbundle By Name(w175) -> ("State"=w176:T4)
        n56 = case shown="\"Repeating\"" w176 {
          tunnel: [_ "Break Continuous" ("State(s) in Front (\"\")") _] -> w172
          frame "Idle" {
            # "The system is already idle. Ignore the \"Stop\" message."
          }
          frame "Repeating" {
            # "If the system is acquiring, stop the acquisition."
          }
          frame "Error" {
          }
        }
        n57 = call <vilib>:"Add State(s) to Queue__JKI_lib_State_Machine.vi"("State(s) in Front (\"\")"=w172, "State(s) in (\"\")"=w174) -> ("States Out"=w173:string)  [unwired: 13 in]
      }
      frame "API: CSM Name" {
        n58 = Bundle By Name(cluster=w179, "CSM Name"=w180) -> (w178:T7)
      }
      frame "API: Steps" {
        n59 = call <vilib>:"Build State String with Arguments__JKI_lib_State_Machine.vi"("Arguments (\"\")"=w183, "State"="Repeat Changed" ("Status with Arguments")) -> ("State with Arguments"=w186:string)  [unwired: 4 in]
        n60 = call <userlib>:"CSM - Broadcast Status Change.vi"("Status With Arguments"=w186, "State Queue"=w185) -> ("Remaining States"=w184:string)  [unwired: 13 in]
      }
      frame "API: INI Read" {
        w191 = T1 [{"控制温度"=25.0, "时长(s)"=60.0, "进度"=1.000390362739563, "温控开关"=FALSE}, {"控制温度"=26.0, "时长(s)"=60.0, "进度"=1.0013926823933919, "温控开关"=TRUE}, {"控制温度"=25.0, "时长(s)"=60.0, "进度"=1.0006222248077392, "温控开关"=FALSE}, {"控制温度"=26.0, "时长(s)"=60.0, "进度"=0.6612281163533529, "温控开关"=TRUE}]  # 循环步骤
        n61 = call "Convert API String Arguments to Data.vim"("Reference Type"=w191, "API String"=w192) -> ("Data"=w190:T1)  [unwired: 6 in, 1 out]
        n62 = local write "步骤"(w190) -> ()
      }
      frame "---------- Repeat ----------" {
        # "#CSM \"Category Seperator\"\nDo not put any code in this frame."
        n63 = call <vilib>:"Add State(s) to Queue__JKI_lib_State_Machine.vi"("State(s) in (\"\")"=w198) -> ("States Out"=w197:string)  [unwired: 14 in]
      }
      frame "Repeat: Initialize" {
        # "#CSM \"Category Seperator\"\nDo not put any code in this frame."
        n64 = Array Size(array="步骤") -> (size(s)=w204:i32)
        n65 = for {
          N: w204 -> [_]
          tunnel: [w208] -> w202 mode=indexing
          i -> [w208]
        }
        n66 = Get Date/Time In Seconds() -> (seconds since 1Jan1904=w203:timestamp)
        n67 = Bundle By Name(cluster=w205, "Repeat.温控步骤开始时间"=w203, "Repeat.温控步骤索引"=w202, "Repeat.下一步？"=TRUE ("下一步？")) -> (w206:T7)
        "当前次数" <- 1 ("当前次数")
      }
      frame "Repeat: Judge" {
        # "#CSM \"Internal State\"\nThis category is used for holding internal states"
        n68 = Unbundle By Name(w215) -> ("State"=w216:T4)
        n69 = case shown="\"Repeating\"" w216 {
          tunnel: [w218 w224 w260] -> w212
          tunnel: w214 -> [w218 w224 w260]
          tunnel: [w217 w229 w259] -> w213
          tunnel: w215 -> [w217 w233 w259]
          tunnel: [_ w220 _] -> w209
          frame "Idle" {
            # "Ignore \"Acquire\" messages when the acquisition is idle."
          }
          frame "Repeating" {
            # "Acquire more data while in the \"Acquiring\" state."
            n70 = Unbundle By Name(w233) -> ("Repeat.温控步骤开始时间"=w247:timestamp, "Repeat.温控步骤索引"=w228:i32[])
            n71 = local read "步骤"() -> (w231:T1)
            n72 = Index Array(array=w228, index=0 ("索引")) -> (element=w239:i32)
            n73 = Index Array(array=w231, index=w239) -> (element=w245:T9)
            n74 = Array Size(array=w228) -> (size(s)=w227:i32)
            n75 = Unbundle By Name(w245) -> ("时长(s)"=w246:dbl)
            n76 = Decrement(x=w227) -> (x-1=w226:i32)
            n77 = Get Date/Time In Seconds() -> (seconds since 1Jan1904=w235:timestamp)
            n78 = local read "当前次数"() -> (w225:i32)
            n79 = Equal?(x=w239, y=w226) -> (x = y?=w241:bool)
            n80 = Subtract(x=w235, y=w247) -> (x-y=w240:dbl)
            n81 = Greater Or Equal?(x=w225, y="运行次数") -> (x >= y?=w244:bool)
            n82 = Greater Or Equal?(x=w240, y=w246) -> (x >= y?=w242:bool)
            n83 = Divide(x=w240, y=w246) -> (x/y=w237:dbl)
            n84 = Compound Arithmetic op=AND ("复合运算")(w242, w241) -> (w243:bool)
            n85 = case shown="True" w242 {
              tunnel: w228 -> [w254 w258]
              tunnel: [w254 w257] -> w238
              tunnel: [FALSE TRUE] -> w219
              frame False {
              }
              frame True {
                n86 = Rotate 1D Array(1:w258, 2:-1 ("n")) -> (0:w257:i32[])
              }
            }
            n87 = case shown="True" w243 {
              tunnel: w244 -> [_ w249]
              tunnel: [_ w248] -> w223
              frame False {
              }
              frame True {
                n88 = case shown="False" w249 {
                  tunnel: [_ TRUE] -> w248
                  frame False {
                    n89 = local read "当前次数"() -> (w250:i32)
                    n90 = Increment(x=w250) -> (x+1=w251:i32)
                    n91 = local write "当前次数"(w251) -> ()
                  }
                  frame True {
                  }
                }
              }
            }
            n92 = Bundle By Name(cluster=w245, "进度"=w237) -> (w236:T9)
            n93 = Replace Array Subset(array=w231, new element=w236, index=w239) -> (w230:T1)
            n94 = Bundle By Name(cluster=w233, "Repeat.温控步骤开始时间"=w247, "Repeat.温控步骤索引"=w238, "Repeat.下一步？"=w219) -> (w229:T7)
            n95 = local write "步骤"(w230) -> ()
            n96 = Select(t="Break Continuous", s=w223, f="Repeat: Func") -> (s? t:f=w220:string)
          }
          frame "Error" {
          }
        }
        n97 = call <vilib>:"Add State(s) to Queue__JKI_lib_State_Machine.vi"("State(s) in Front (\"\")"=w209, "State(s) in (\"\")"=w210) -> ("States Out"=w211:string)  [unwired: 13 in]
      }
      frame "Repeat: Func" {
        n98 = Unbundle By Name(w269) -> ("CSM Name"=w263:string, "Repeat.下一步？"=w282:bool, "Repeat.温控步骤索引"=w278:i32[], "Repeat.温控步骤开始时间"=w274:timestamp)
        n99 = local read "步骤"() -> (w267:T1)
        n100 = Index Array(array=w278, index=0 ("索引")) -> (element=w279:i32)
        n101 = feedback #1(-1 ("索引")) -> (w273:i32)
        n102 = feedback-in #1(w279) -> ()
        n103 = Index Array(array=w267, index=w279) -> (element=w277:T9)
        n104 = Not Equal?(x=w279, y=w273) -> (x != y?=w281:bool)
        n105 = Unbundle By Name(w277) -> ("控制温度"=w276:dbl, "温控开关"=w280:bool)
        n106 = Compound Arithmetic op=OR ("复合运算")(w282, w281) -> (w261:bool)
        n107 = case shown="True" w261 {
          tunnel: w280 -> [_ w289]
          tunnel: w276 -> [_ w288]
          tunnel: "通道选择" -> [_ w287]
          tunnel: w263 -> [_ w286]
          tunnel: ["" ("States Out") w285] -> w262
          frame False {
          }
          frame True {
            n108 = case shown="\"1\", 默认" w287 {
              tunnel: w288 -> [w298 w304 w323]
              tunnel: w289 -> [w299 w303 w324]
              tunnel: w286 -> [w293 w305 w317]
              tunnel: [w292 w302 w313] -> w285
              frame "1", Default {
                n109 = call "Convert Data To API String Arguments.vim"("Data"=w298) -> ("API String"=w295:string)  [unwired: 7 in, 1 out]
                n110 = call "Convert Data To API String Arguments.vim"("Data"=w299) -> ("API String"=w290:string)  [unwired: 7 in, 1 out]
                n111 = call-poly <userlib>:"Build Message with Arguments++.vi"("State With Arguments"="Action: Power Output 1", "Arguments (\"\")"=w290, "Target Module (\"\")"=w293) -> ("CSM Message String"=w297:string)  [unwired: 12 in]
                n112 = call-poly <userlib>:"Build Message with Arguments++.vi"("State With Arguments"="Action: Change Temp 1", "Arguments (\"\")"=w295, "Target Module (\"\")"=w293) -> ("CSM Message String"=w294:string)  [unwired: 12 in]
                n113 = call <vilib>:"Add State(s) to Queue__JKI_lib_State_Machine.vi"("State(s) in Front (\"\")"=w294, "State(s) in (\"\")"=w297) -> ("States Out"=w292:string)  [unwired: 13 in]
              }
              frame "2" {
                n114 = call "Convert Data To API String Arguments.vim"("Data"=w304) -> ("API String"=w307:string)  [unwired: 7 in, 1 out]
                n115 = call "Convert Data To API String Arguments.vim"("Data"=w303) -> ("API String"=w300:string)  [unwired: 7 in, 1 out]
                n116 = call-poly <userlib>:"Build Message with Arguments++.vi"("State With Arguments"="Action: Power Output 2", "Arguments (\"\")"=w300, "Target Module (\"\")"=w305) -> ("CSM Message String"=w309:string)  [unwired: 12 in]
                n117 = call-poly <userlib>:"Build Message with Arguments++.vi"("State With Arguments"="Action: Change Temp 2", "Arguments (\"\")"=w307, "Target Module (\"\")"=w305) -> ("CSM Message String"=w306:string)  [unwired: 12 in]
                n118 = call <vilib>:"Add State(s) to Queue__JKI_lib_State_Machine.vi"("State(s) in Front (\"\")"=w306, "State(s) in (\"\")"=w309) -> ("States Out"=w302:string)  [unwired: 13 in]
              }
              frame "1&2" {
                n119 = call "Convert Data To API String Arguments.vim"("Data"=w323) -> ("API String"=w318:string)  [unwired: 7 in, 1 out]
                n120 = call "Convert Data To API String Arguments.vim"("Data"=w324) -> ("API String"=w310:string)  [unwired: 7 in, 1 out]
                n121 = call-poly <userlib>:"Build Message with Arguments++.vi"("State With Arguments"="Action: Power Output 1", "Arguments (\"\")"=w310, "Target Module (\"\")"=w317) -> ("CSM Message String"=w322:string)  [unwired: 12 in]
                n122 = call-poly <userlib>:"Build Message with Arguments++.vi"("State With Arguments"="Action: Change Temp 1", "Arguments (\"\")"=w318, "Target Module (\"\")"=w317) -> ("CSM Message String"=w320:string)  [unwired: 12 in]
                n123 = call <vilib>:"Add State(s) to Queue__JKI_lib_State_Machine.vi"("State(s) in Front (\"\")"=w320, "State(s) in (\"\")"=w322) -> ("States Out"=w314:string)  [unwired: 13 in]
                n124 = call-poly <userlib>:"Build Message with Arguments++.vi"("State With Arguments"="Action: Power Output 2", "Arguments (\"\")"=w310, "Target Module (\"\")"=w317) -> ("CSM Message String"=w315:string)  [unwired: 12 in]
                n125 = call-poly <userlib>:"Build Message with Arguments++.vi"("State With Arguments"="Action: Change Temp 2", "Arguments (\"\")"=w318, "Target Module (\"\")"=w317) -> ("CSM Message String"=w316:string)  [unwired: 12 in]
                n126 = call <vilib>:"Add State(s) to Queue__JKI_lib_State_Machine.vi"("State(s) in Front (\"\")"=w314, "State(s) in (\"\")"=w316, "State(s) at Back (\"\")"=w315) -> ("States Out"=w313:string)  [unwired: 12 in]
              }
            }
          }
        }
        n127 = case shown="True" w281 {
          tunnel: [w325 w326] -> w275
          tunnel: w274 -> [w325 _]
          frame False {
          }
          frame True {
            n128 = Get Date/Time In Seconds() -> (seconds since 1Jan1904=w326:timestamp)
          }
        }
        n129 = Bundle By Name(cluster=w269, "Repeat.下一步？"=FALSE ("下一步？"), "Repeat.温控步骤开始时间"=w275) -> (w268:T7)
        n130 = call <vilib>:"Add State(s) to Queue__JKI_lib_State_Machine.vi"("State(s) in Front (\"\")"=w262, "State(s) in (\"\")"=w264) -> ("States Out"=w265:string)  [unwired: 13 in]
      }
      frame "Repeat: Stop" {
        # "#CSM \"Internal State\"\nThis category is used for holding internal states"
        n131 = local write "循环开始"(FALSE ("循环开始")) -> ()
        n132 = call <vilib>:"Add State(s) to Queue__JKI_lib_State_Machine.vi"("State(s) in (\"\")"=w330) -> ("States Out"=w329:string)  [unwired: 14 in]
      }
      frame "Repeat: Close" {
        w331 = Repeating_States."Idle"  # State
        # "#CSM \"Internal State\"\nThis category is used for holding internal states"
        n133 = Bundle By Name(cluster=w333, "State"=w331) -> (w332:T7)
        n134 = call <vilib>:"Add State(s) to Queue__JKI_lib_State_Machine.vi"("State(s) in (\"\")"=w335) -> ("States Out"=w334:string)  [unwired: 14 in]
      }
      frame "---------- Loop ----------" {
        # "#CSM \"Internal State\"\nThis category is used for holding internal states"
        n135 = call <vilib>:"Add State(s) to Queue__JKI_lib_State_Machine.vi"("State(s) in (\"\")"=w338) -> ("States Out"=w337:string)  [unwired: 14 in]
      }
      frame "Continuous Check" {
        # "#CSM \"Internal State\"\nThis category is used for holding internal states"
        n136 = Wait (ms)(milliseconds to wait=u32 75 ("等待时间（毫秒）")) -> ()  [unwired: 1 out]
        n137 = call <userlib>:"CSMLS - Append Continuous State.vi"("Loop State(s) And Arguments"=w340, "Continous Arguments (\"\")"=w340, "Continous State"=w342, "States Queue"=w343) -> ("Remaining States"=w341:string)  [unwired: 7 in]
      }
      frame "Break Continuous" {
        n138 = call <userlib>:"CSMLS - Remove Loop Tag to Break.vi"("States Queue"=w347) -> ("Remaining States"=w345:string)  [unwired: 10 in]
      }
    }
  }
  n139 = while {
    shift-right: [w359] -> _
    shift-left: enum16{"Idle", "Initialize", "Exit"}."Initialize" -> [w360]
    tunnel: "CSM Name" -> [w357]
    shift-right: [w355] -> _
    shift-left: w5 -> [w356]
    shift-right: [w353] -> _
    shift-left: -1 -> [w354]
    shift-right: [w352] -> _
    shift-left: _ -> [w351]
    shift-right: [w350] -> _
    shift-left: _ -> [w349]
    stop <- w358 stop-if-true
    n140 = case shown="\"Idle\", 默认" w360 {
      tunnel: [enum16{"Idle", "Initialize", "Exit"}."Idle" w378 enum16{"Idle", "Initialize", "Exit"}."Exit"] -> w359
      tunnel: [_ _ TRUE] -> w358
      tunnel: w357 -> [w364 w377 _]
      tunnel: w356 -> [w367 w375 w405]
      tunnel: [w367 w376 w405] -> w355
      tunnel: w354 -> [_ w373 _]
      tunnel: [-1 w374 _] -> w353
      tunnel: [w363 w371 _] -> w352
      tunnel: w351 -> [_ w372 w404]
      tunnel: [w361 w369 w402] -> w350
      tunnel: w349 -> [_ w370 w402]
      frame "Initialize" {
        w362 = FALSE  # your data
        n141 = call <userlib>:"CSM - Module Exit Event.vi"("Name (\"\" to Use UUID) In"=w364) -> ("CSM Exit Event"=w365:refnum<user-event>)  [unwired: 8 in, 2 out]
        n142 = register-events(w365) -> (reference out=w363:refnum<event-registration>)  [unwired: 2 in, 1 out]
        n143 = Bundle("your data"=w362) -> (w361:cluster{"your data":bool})  [unwired: 1 in]
      }
      frame "Idle", Default {
        n144 = event shown="[2] \"循环开始\": 值改变" {
          selector: w372 -> [_ _ _ _]
          dyn-events: [_ _ _ _] -> w371
          timeout: w373 -> [_ _ _ _]
          tunnel: [_ enum16{"Idle", "Initialize", "Exit"}."Exit" _ _] -> w378
          tunnel: w377 -> [w380 _ _ _]
          tunnel: w375 -> [w383 w387 w392 w399]
          tunnel: [w381 w387 w393 w400] -> w376
          tunnel: [-1 _ _ _] -> w374
          tunnel: w370 -> [w379 w385 w394 w401]
          tunnel: [w379 w385 w394 w401] -> w369
          event Timeout {
            n145 = event-data() -> ()  [unwired: 1 in, 3 out]
            n146 = call-poly <userlib>:"CSM - Filter JKISM String Queue.vi"("States In"=w383) -> ("States Out"=w382:string)  [unwired: 14 in]
            n147 = call <userlib>:"CSM - Forward UI Operations to CSM.vi"("Name (\"\" to Use UUID)"=w380, "State(s) In (\"\")"=w382) -> ("States Out"=w381:string)  [unwired: 8 in, 1 out]
          }
          event User Event {
            n148 = event-data() -> ()  [unwired: 1 in, 1 out]
          }
          event "循环开始": Value Change {
            n149 = event-data() -> ()  [unwired: 1 in, 1 out]
            n150 = Select(t="API: Start", s="循环开始", f="API: Stop") -> (s? t:f=w388:string)
            n151 = call <vilib>:"Add State(s) to Queue__JKI_lib_State_Machine.vi"("State(s) in Front (\"\")"=w388, "State(s) in (\"\")"=w392) -> ("States Out"=w393:string)  [unwired: 13 in]
          }
          event Value Change {
            n152 = event-data() -> ("NewVal"=w398:T1)  [unwired: 1 in]
            n153 = call "Convert Data To API String Arguments.vim"("Data"=w398) -> ("API String"=w397:string)  [unwired: 7 in, 1 out]
            n154 = call <vilib>:"Build State String with Arguments__JKI_lib_State_Machine.vi"("Arguments (\"\")"=w397, "State"="API: Steps") -> ("State with Arguments"=w395:string)  [unwired: 4 in]
            n155 = call <vilib>:"Add State(s) to Queue__jki_lib_state_machine.vi"("State(s) in Front (\"\")"=w395, "State(s) in (\"\")"=w399) -> ("States Out"=w400:string)  [unwired: 13 in]
          }
        }
      }
      frame "Exit" {
        n156 = Unregister For Events(event registration refnum=w404) -> (error out=w403:errorcluster)  [unwired: 1 in]
        n157 = call <vilib>:"Clear Errors.vi"("error in (no error)"=w403) -> ()  [unwired: 5 in, 2 out]
      }
    }
  }
  n158 = call <userlib>:"CSM - Sync Configuration Variables to File.vi"("All Temp Variable to Default Ini(F)"=TRUE, "error in (no error)"=w2) -> ()  [unwired: 7 in, 1 out]
